vi "Commentaire Logbook.vi"() -> ()   [LabVIEW 2022 SP3]
uses:
  Enum/Enum 10.ctl
  Variables globales/Variable glob generale.vi
panel:
  out "Dernier commentaire enregistré":string
  out "référence en sortie":refnum<vi>
  in  "Sortir":bool
  out "à enregistrer":string
  in  "Date et heure":bool
  in  "Choix date et heure":timestamp format="%<%X\n%x>T"
  in  "Bouton OK":bool
  in  "Commentaire":string
  out "Temps actuel":timestamp format="%<%X\n%x>T"
  # "insertion commentaire\ndans fichier logbook"
  # "Ce logiciel et les informations qu'il contient, sont la propriété de l’IAS et ne peuvent être diffusés sans l’autorisation de la Station d’étalonnage"
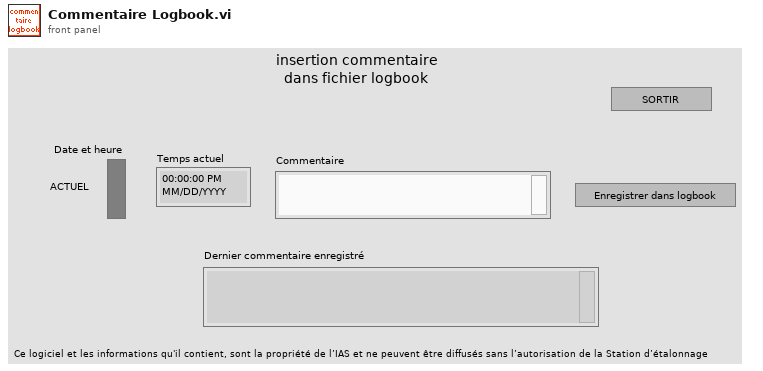
[diagram p1: front panel]
types:
  T1 = typedef "Enum 10.ctl" = enum16{"init", "attente", "chaine", "message", "écriture", "RAZ", "fin"}
  T2 = enum32{"Invalid", "Standard", "Closed", "Hidden", "Minimized", "Maximized"}
  T3 = enum16{"open", "replace", "create", "open or create", "replace or create", "replace or create with confirmation"}
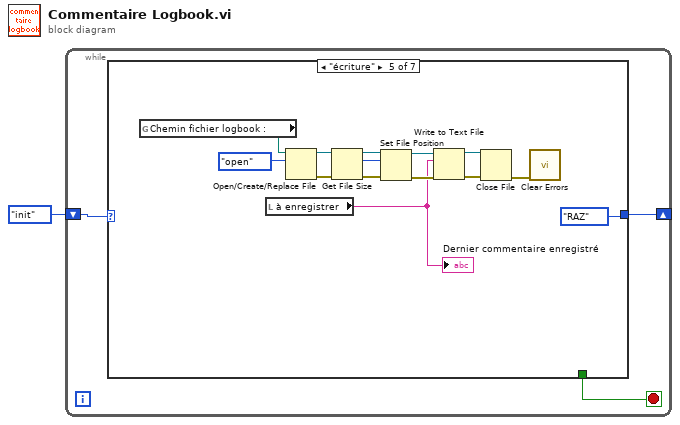
[diagram p0: block diagram]
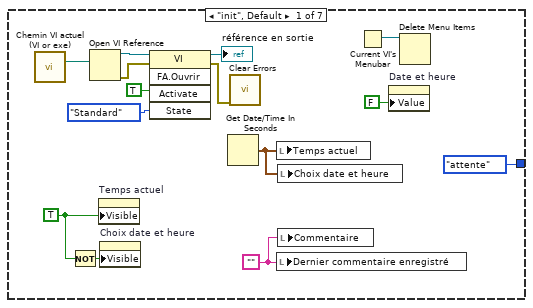
[diagram p2: hidden frame]
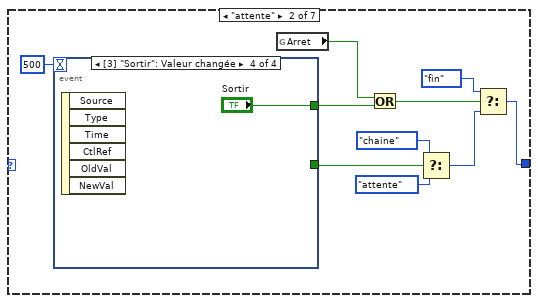
[diagram p3: hidden frame]
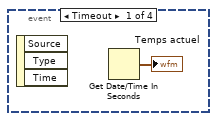
[diagram p4: hidden frame]
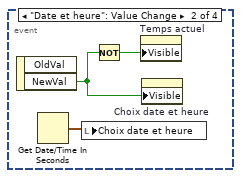
[diagram p5: hidden frame]
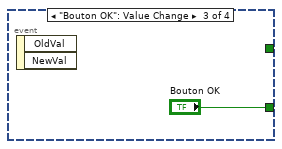
[diagram p6: hidden frame]
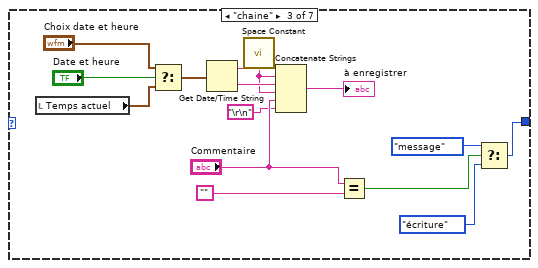
[diagram p7: hidden frame]
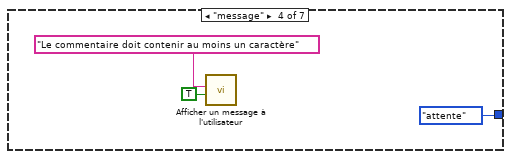
[diagram p8: hidden frame]
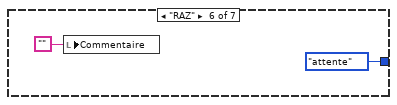
[diagram p9: hidden frame]
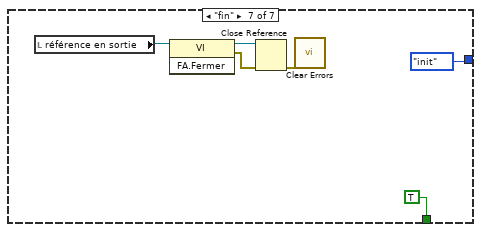
[diagram p10: hidden frame]
diagram:
  n1 = while {
    shift-right: [w3] -> _
    shift-left: Enum_10."init" ("Énum") -> [w4]
    stop <- w2 stop-if-true
    n2 = case shown="\"écriture\"" w4 {
      tunnel: [Enum_10."attente" ("Énum") w22 w40 Enum_10."attente" ("Énum") Enum_10."RAZ" ("Énum") Enum_10."attente" ("Énum") Enum_10."init" ("Énum")] -> w3
      tunnel: [_ _ _ _ _ _ TRUE] -> w2
      frame "init", Default {
        w5 = ""
        w6 = TRUE ("Visible")
        n3 = call "Chemin VI actuel (VI or exe).vi"() -> ("Full Path to VI or executable"=w16:path)  [unwired: 14 in, 1 out]
        n4 = Not(x=w6) -> (.not. x?=w8:bool)
        n5 = Open VI Reference(vi path=w16) -> (vi reference=w12:refnum<vi>, error out=w14:errorcluster)  [unwired: 5 in]
        n6 = property on="Temps actuel" class="TempsAbs (strict)"("Visible"=w6) -> ()  [unwired: 2 in, 2 out]
        n7 = property on="Choix date et heure" class="TempsAbs (strict)"("Visible"=w8) -> ()  [unwired: 2 in, 2 out]
        n8 = invoke class="VI" method="FA.Ouvrir"(reference=w12, error in=w14, "Activate"=TRUE ("Activer ?"), "State"=T2."Standard" ("État")) -> (reference out=→"référence en sortie":refnum<vi>, error out=w15:errorcluster)  [unwired: 1 in, 3 out]
        n9 = Get Date/Time In Seconds() -> (seconds since 1Jan1904=w7:timestamp)
        n10 = call <vilib>:"Clear Errors.vi"("error in (no error)"=w15) -> ()  [unwired: 5 in, 2 out]
        n11 = local write "Temps actuel"(w7) -> ()
        n12 = local write "Dernier commentaire enregistré"(w5) -> ()
        n13 = local write "Choix date et heure"(w7) -> ()
        n14 = local write "Commentaire"(w5) -> ()
        n15 = Current VI's Menubar() -> (w18:refnum<k9>)
        n16 = property on="Date et heure" class="Bool (strict)"("Value"=FALSE ("Date et heure")) -> ()  [unwired: 2 in, 2 out]
        n17 = Delete Menu Items(9:w18) -> ()  [unwired: 3 in, 2 out]
      }
      frame "attente" {
        n18 = event shown="[3] \"Sortir\": Valeur changée" {
          selector: _ -> [_ _ _ _]
          dyn-events: _ -> [_ _ _ _]
          timeout: 500 -> [_ _ _ _]
          tunnel: [_ _ "Bouton OK" _] -> w27
          tunnel: [_ _ _ "Sortir"] -> w20
          event Timeout {
            n19 = event-data() -> ()  [unwired: 1 in, 3 out]
            n20 = Get Date/Time In Seconds() -> (seconds since 1Jan1904=→"Temps actuel":timestamp)
          }
          event "Date et heure": Value Change {
            n21 = event-data() -> ("NewVal"=w32:bool)  [unwired: 1 in, 1 out]
            n22 = Get Date/Time In Seconds() -> (seconds since 1Jan1904=w30:timestamp)
            n23 = local write "Choix date et heure"(w30) -> ()
            n24 = Not(x=w32) -> (.not. x?=w31:bool)
            n25 = property on="Temps actuel" class="TempsAbs (strict)"("Visible"=w31) -> ()  [unwired: 2 in, 2 out]
            n26 = property on="Choix date et heure" class="TempsAbs (strict)"("Visible"=w32) -> ()  [unwired: 2 in, 2 out]
          }
          event "Bouton OK": Value Change {
            n27 = event-data() -> ()  [unwired: 1 in, 2 out]
          }
          event "Sortir": Value Change {
            n28 = event-data() -> ()  [unwired: 1 in, 6 out]
          }
        }
        n29 = global read "Variable glob generale.vi" "Arret"() -> (w21:bool)
        n30 = Or(x=w21, y=w20) -> (x .or. y?=w19:bool)
        n31 = Select(t=Enum_10."chaine" ("Énum"), s=w27, f=Enum_10."attente" ("Énum")) -> (s? t:f=w23:T1)
        n32 = Select(t=Enum_10."fin" ("Énum"), s=w19, f=w23) -> (s? t:f=w22:T1)
      }
      frame "chaine" {
        n33 = local read "Temps actuel"() -> (w46:timestamp)
        n34 = Select(t="Choix date et heure", s="Date et heure", f=w46) -> (s? t:f=w44:timestamp)
        n35 = Get Date/Time String(seconds (now)=w44) -> (date string=w49:string, time string=w48:string)  [unwired: 2 in]
        n36 = call <vilib>:"Space Constant.vi"() -> ("String"=w38:string)
        n37 = Concatenate Strings(w49, w38, w48, w38, "Commentaire", "\r\n") -> (→"à enregistrer":string)
        n38 = Equal?(x="Commentaire", y="") -> (x = y?=w42:bool)
        n39 = Select(t=Enum_10."message" ("Énum"), s=w42, f=Enum_10."écriture" ("Énum")) -> (s? t:f=w40:T1)
      }
      frame "message" {
        n40 = call "Afficher un message à l'utilisateur"("Enable"=TRUE, "Message"="Le commentaire doit contenir au moins un caractère") -> ()  [unwired: 8 in, 2 out]
      }
      frame "écriture" {
        n41 = global read "Variable glob generale.vi" "Chemin fichier logbook :"() -> (w65:path)
        n42 = local read "à enregistrer"() -> (w53:string)
        "Dernier commentaire enregistré" <- w53
        n43 = Open/Create/Replace File(file path (use dialog)=w65, operation (0:open)=T3."open" ("opération (0 : open)")) -> (refnum out=w60:refnum<file>, error out=w59:errorcluster)  [unwired: 1 in, 4 out]
        n44 = Get File Size(file=w60, error in=w59) -> (refnum out=w56:refnum<file>, size (in bytes)=w57:i64, 0:w58:errorcluster)
        n45 = Set File Position(offset (in bytes) (0)=w57, refnum=w56, error in=w58) -> (refnum out=w55:refnum<file>, error out=w54:errorcluster)  [unwired: 1 in]
        n46 = Write to Text File(file (use dialog)=w55, text=w53, error in=w54) -> (refnum out=w63:refnum<file>, error out=w62:errorcluster)  [unwired: 1 in, 1 out]
        n47 = Close File(refnum=w63, error in=w62) -> (error out=w64:errorcluster)  [unwired: 1 out]
        n48 = call <vilib>:"Clear Errors.vi"("error in (no error)"=w64) -> ()  [unwired: 5 in, 2 out]
      }
      frame "RAZ" {
        n49 = local write "Commentaire"("") -> ()
      }
      frame "fin" {
        n50 = local read "référence en sortie"() -> (w69:refnum<vi>)
        n51 = invoke class="VI" method="FA.Fermer"(reference=w69) -> (reference out=w71:refnum<vi>, error out=w70:errorcluster)  [unwired: 2 in, 1 out]
        n52 = Close Reference(reference=w71, error in (no error)=w70) -> (error out=w72:errorcluster)
        n53 = call <vilib>:"Clear Errors.vi"("error in (no error)"=w72) -> ()  [unwired: 5 in, 2 out]
      }
    }
  }
